vi "UIHandlerMain.vi"(6 "timeout_ms":i32=100, 8 "error in":errorcluster, 11 "UI_Manager in":refnum<class "UI_Library.lvclass">) -> (0 "error out":errorcluster, 1 "data":variant, 2 "cmd":string, 3 "UI_Manager out":refnum<class "UI_Library.lvclass">, 4 "CloseUILoop":bool, 5 "#el_queue":i32)   [LabVIEW 2025, in "UI_Library.lvlib" / "UI_Library.lvclass"]
doc: "Update UI in accordance to the message received"
uses:
  UI_Library.lvclass
  UI_Library.lvclass/UI_Library.ctl
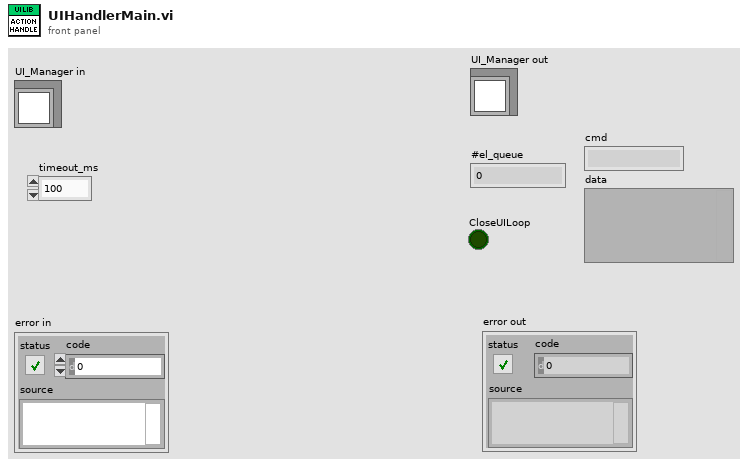
[diagram p1: front panel]
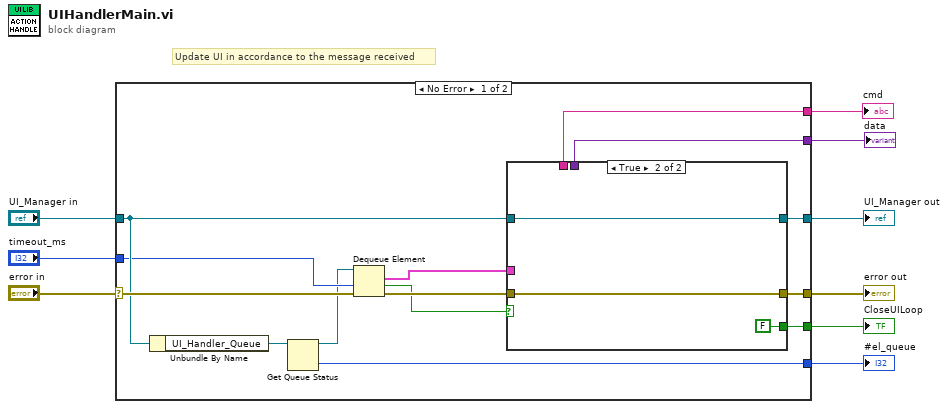
[diagram p0: block diagram]
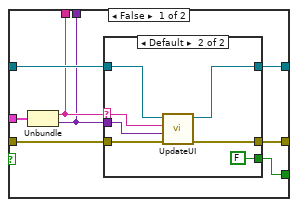
[diagram p2: hidden frame]
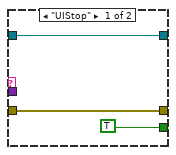
[diagram p3: hidden frame]
diagram:
  # "Update UI in accordance to the message received"
  n1 = case shown="No Error" "error in" {
    selector: "error in" -> [w23 w45]
    tunnel: "UI_Manager in" -> [w22 w46]
    tunnel: [w21 w46] -> w7
    tunnel: [w20 w45] -> w6
    tunnel: "timeout_ms" -> [w19 _]
    tunnel: [w18 _] -> w4
    tunnel: [w12 _] -> w3
    tunnel: [w11 _] -> w2
    tunnel: [w10 _] -> w1
    frame No Error {
      n2 = Unbundle By Name(w22) -> ("UI_Handler_Queue"=w17:refnum<queue>)
      n3 = Get Queue Status(queue=w17) -> (queue out=w13:refnum<queue>, # elements in queue=w18:i32)  [unwired: 2 in, 6 out]
      n4 = Dequeue Element(queue=w13, timeout in ms (-1)=w19, error in (no error)=w23) -> (element=w16:cluster{"cmd":string, "data":variant}, timed out?=w14:bool, error out=w15:errorcluster)  [unwired: 1 out]
      n5 = case shown="True" w14 {
        tunnel: w16 -> [w31 _]
        tunnel: w15 -> [w30 w43]
        tunnel: w22 -> [w29 w44]
        tunnel: [w28 w44] -> w21
        tunnel: [w27 w43] -> w20
        tunnel: [w26 FALSE] -> w12
        tunnel: [w25 _] -> w11
        tunnel: [w24 _] -> w10
        frame False {
          n6 = Unbundle(w31) -> ("cmd"=w25:string, "data"=w24:variant)
          n7 = case shown="Default" w25 {
            selector: w25 -> [_ w41]
            tunnel: w24 -> [_ w40]
            tunnel: w30 -> [w34 w39]
            tunnel: w29 -> [w33 w38]
            tunnel: [w33 w37] -> w28
            tunnel: [w34 w36] -> w27
            tunnel: [TRUE FALSE] -> w26
            frame "UIStop" {
            }
            frame Default {
              n8 = call-dynamic "UpdateUI.vi"("error in"=w39, "Control Data"=w40, "Action"=w41, "UI_Manager in"=w38) -> ("error out"=w36:errorcluster, "UI_Manager out"=w37:refnum<class "UI_Library.lvclass">)  [unwired: 6 in]
            }
          }
        }
        frame True {
        }
      }
    }
    frame Error {
    }
  }
  "UI_Manager out" <- w7
  "error out" <- w6
  "#el_queue" <- w4
  "CloseUILoop" <- w3
  "cmd" <- w2
  "data" <- w1
